vi "test Get-Set-Get Label Properties.vi"(8 "error in":errorcluster, 11 "TestCase in":refnum<class "Scripting.lvclass">) -> (0 "error out":errorcluster, 3 "TestCase out":refnum<class "Scripting.lvclass">)   [LabVIEW 2020, in "Scripting.lvclass"]
uses:
  Scripting.lvclass
  Shared/Label Properties.ctl
  Scripting.lvclass/Scripting.ctl
  <vilib>/addons/_JKI Toolkits/VI Tester/TestCase.llb/TestCase.lvclass
  Scripting/Ballard/Ballard ARINC 429 Scripting.lvlib
  Scripting/ARINC 429/ARINC 429 Scripting.lvlib
  Shared/Label.ctl
  C:/Program Files (x86)/National Instruments/LabVIEW 2020/vi.lib/addons/_JKI Toolkits/VI Tester/TestCase.llb/TestCase.lvclass
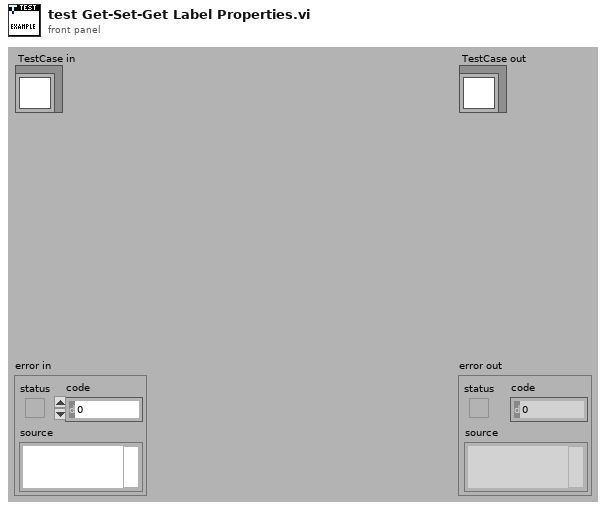
[diagram p1: front panel]
types:
  T1 = typedef "Label Properties.ctl" = cluster{"label (Dec)":T2, "SDI value":u8, "SDI enabled":bool}
  T2 = typedef "Label.ctl" = u8
  T3 = typedef "Custom Device API.lvlib/Custom Device Item Ref.ctl" = u64
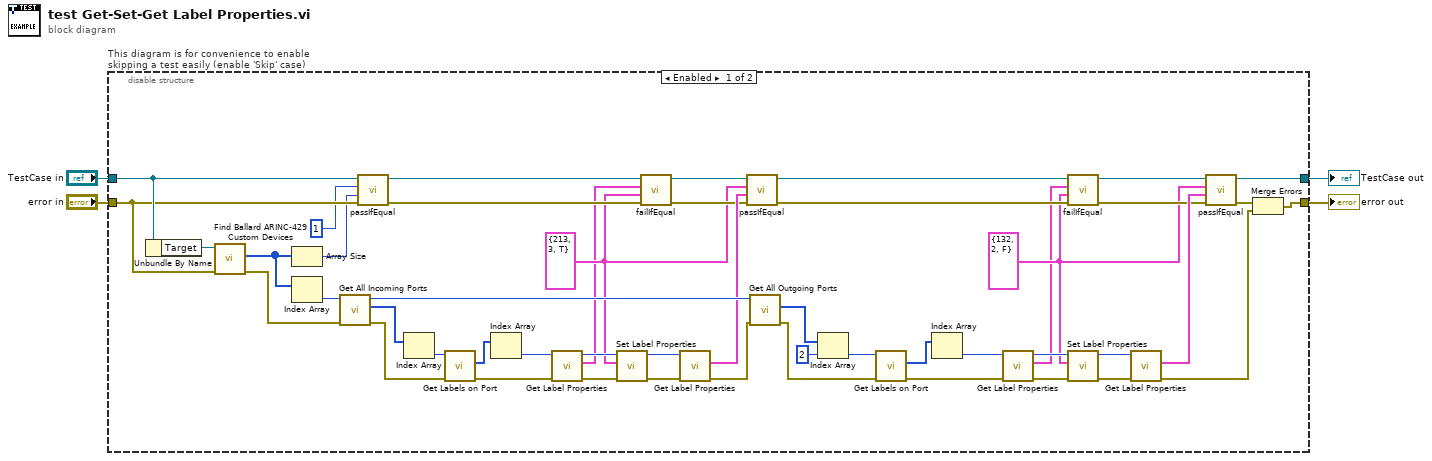
[diagram p0: block diagram]
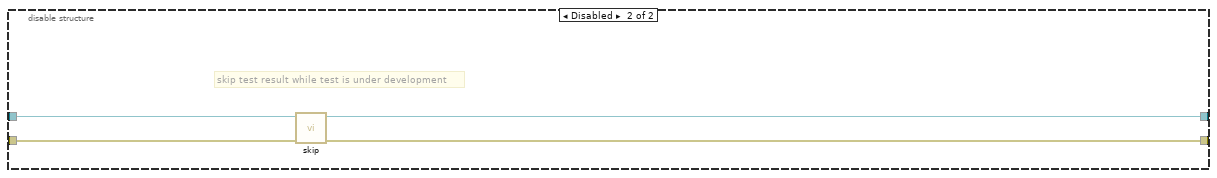
[diagram p2: hidden frame]
diagram:
  n1 = disable-structure "This diagram is for convenience to enable skipping a test easily (enable 'Skip' case)" shown="Enabled" {
    disable-tunnel: "TestCase in" -> [w51 w57]
    disable-tunnel: [w34 w55] -> w1
    disable-tunnel: [w42 w56] -> w3
    disable-tunnel: "error in" -> [w50 w54]
    frame Enabled {
      w7 = T1 {"label (Dec)"=132, "SDI value"=2, "SDI enabled"=FALSE} ("label properties")
      w13 = T1 {"label (Dec)"=213, "SDI value"=3, "SDI enabled"=TRUE} ("label properties")
      n2 = Unbundle By Name(w51) -> ("Target"=w53:refnum<k24>)
      n3 = call "Find Ballard ARINC-429 Custom Devices.vi"("error in"=w50, "target in"=w53) -> ("error out"=w46:errorcluster, "Ballard ARINC 429 custom devices"=w5:u64[])  [unwired: 7 in, 1 out]
      n4 = Array Size(array=w5) -> (size(s)=w48:i32)
      n5 = Index Array(array=w5) -> (element=w52:u64)  [unwired: 1 in]
      n6 = call "Get All Incoming Ports.vi"("error in"=w46, "Ballard ARINC 429 ref"=w52) -> ("error out"=w40:errorcluster, "Port refs"=w47:T3[], "Ballard ARINC 429 ref out"=w45:T3)  [unwired: 7 in]
      n7 = call-dynamic "passIfEqual.vi"("error in (no error)"=w50, "y"=w48, "x"=1 ("size(s)"), "TestCase in"=w51) -> ("error out"=w16:errorcluster, "TestCase out"=w17:refnum<class "Scripting.lvclass">)  [unwired: 6 in]
      n8 = Index Array(array=w47) -> (element=w41:T3)  [unwired: 1 in]
      n9 = call "Get Labels on Port.vi"("error in"=w40, "port ref"=w41) -> ("error out"=w28:errorcluster, "label references"=w36:T3[])  [unwired: 6 in, 2 out]
      n10 = Index Array(array=w36) -> (element=w29:T3)  [unwired: 1 in]
      n11 = call "Get Label Properties.vi"("error in"=w28, "label ref in"=w29) -> ("error out"=w32:errorcluster, "label properties"=w12:T1, "label ref out"=w33:T3)  [unwired: 6 in, 1 out]
      n12 = call "Set Label Properties.vi"("error in"=w32, "label properties"=w13, "label ref"=w33) -> ("error out"=w30:errorcluster, "label ref out"=w31:T3)  [unwired: 7 in]
      n13 = call-dynamic "failIfEqual.vi"("error in (no error)"=w16, "y"=w13, "x"=w12, "TestCase in"=w17) -> ("error out"=w14:errorcluster, "TestCase out"=w15:refnum<class "Scripting.lvclass">)  [unwired: 6 in]
      n14 = call "Get Label Properties.vi"("error in"=w30, "label ref in"=w31) -> ("error out"=w27:errorcluster, "label properties"=w26:T1)  [unwired: 6 in, 2 out]
      n15 = call-dynamic "passIfEqual.vi"("error in (no error)"=w14, "y"=w26, "x"=w13, "TestCase in"=w15) -> ("error out"=w10:errorcluster, "TestCase out"=w11:refnum<class "Scripting.lvclass">)  [unwired: 6 in]
      n16 = call "Get All Outgoing Ports.vi"("error in"=w27, "Ballard ARINC 429 ref"=w45) -> ("error out"=w39:errorcluster, "Port refs"=w44:T3[])  [unwired: 7 in, 1 out]
      n17 = Index Array(array=w44, index=2) -> (element=w38:T3)
      n18 = call "Get Labels on Port.vi"("error in"=w39, "port ref"=w38) -> ("error out"=w20:errorcluster, "label references"=w37:T3[])  [unwired: 6 in, 2 out]
      n19 = Index Array(array=w37) -> (element=w21:T3)  [unwired: 1 in]
      n20 = call "Get Label Properties.vi"("error in"=w20, "label ref in"=w21) -> ("error out"=w23:errorcluster, "label properties"=w6:T1, "label ref out"=w22:T3)  [unwired: 6 in, 1 out]
      n21 = call-dynamic "failIfEqual.vi"("error in (no error)"=w10, "y"=w7, "x"=w6, "TestCase in"=w11) -> ("error out"=w8:errorcluster, "TestCase out"=w9:refnum<class "Scripting.lvclass">)  [unwired: 6 in]
      n22 = call "Set Label Properties.vi"("error in"=w23, "label properties"=w7, "label ref"=w22) -> ("error out"=w25:errorcluster, "label ref out"=w24:T3)  [unwired: 7 in]
      n23 = call "Get Label Properties.vi"("error in"=w25, "label ref in"=w24) -> ("error out"=w19:errorcluster, "label properties"=w18:T1)  [unwired: 6 in, 2 out]
      n24 = call-dynamic "passIfEqual.vi"("error in (no error)"=w8, "y"=w18, "x"=w7, "TestCase in"=w9) -> ("error out"=w35:errorcluster, "TestCase out"=w34:refnum<class "Scripting.lvclass">)  [unwired: 6 in]
      n25 = Merge Errors(w35, w19) -> (w42:errorcluster)
    }
    frame Disabled {
      # "skip test result while test is under development"
      n26 = call <vilib>:"skip.vi"("error in (no error)"=w54, "TestCase in"=w57) -> ("error out"=w56:errorcluster, "TestCase out"=w55:refnum<class "Scripting.lvclass">)  [unwired: 8 in]
    }
  }
  "error out" <- w3
  "TestCase out" <- w1
